vi "DepthProfiling_Proc.vi"(5 "DP_filepath":path=path "", 7 "Params.":variant, 8 "error in (no error)":errorcluster, 9 "Dynamic Params In":refnum<queue>, 10 "Quit_UserEvent":refnum<user-event>, 11 "ControlQueueRef":variant) -> (0 "error out":errorcluster, 2 "Output":variant)   [LabVIEW 2013]
uses:
  Apps_static/ScanParams_SingleLine.ctl
  ProcessMethods/Binning/BinType.ctl
  Files/BinaryHeader.ctl
  ControlDef/QueueRefs.ctl
  ControlDef/LaserCtrl_Method.ctl
  ControlDef/States-AToF.ctl
  <instrlib>/AnalogDiscSDKLv/VIs/DWF_CtrlQueue.ctl
  <instrlib>/AnalogDiscSDKLv/VIs/DWF_State.ctl
  <instrlib>/ESP300/Public/Data/ESP300_State.ctl
  <instrlib>/DG535/Command/DG535_States.ctl
  Hardware/BNC(QuantumComposers)/BNC_States.ctl
  Hardware/FemtoLaser(Legacy)/Laser_Status.ctl
  Hardware/DAQmx(Legacy)/DAQmx_Status.ctl
  ControlDef/Signal.ctl
  ProcessMethods/SignalAverager/ProcessStates.ctl
  Files/WriterState.ctl
  Files/Signal_Segment.ctl
  ControlDef/ProcessingMode.ctl
  Hardware/EPM2000(Legacy)/EPM2K_Status.ctl
  <instrlib>/AnalogDiscSDKLv/VIs/DWF_Signal.ctl
  ControlDef/SampleRateSelector.ctl
  ImagingMS/DirectImaging_State.ctl
  ImagingMS/Imaging_Params.ctl
  ProcessMethods/BioMapConversion/BioMAPWriterCoreParams.ctl
  <vilib>/Utility/error.llb/DialogType.ctl
  <vilib>/Utility/miscctls.llb/LVRowAndColumnTypeDef.ctl
  <vilib>/Analysis/baseanly.llb/Mean (DBL).vi
  UI/Autoscale_Y_Single.vi
  <userlib>/_OpenG.lib/comparison/comparison.llb/I32 Changed__ogtk.vi
  ProcessMethods/Binning/SpectrumBinning.vi
  <instrlib>/ESP300/ESP300.lvlib
  <instrlib>/DG535/SRS_DG535_Lib.lvlib
  <userlib>/Utility/ErrorLog_lib.lvlib
  <vilib>/Analysis/NI_AALBase.lvlib
  <instrlib>/AnalogDiscSDKLv/AnalogDiscSDKLv.lvlib
panel:
  in  "SaveMiddleFile":bool
  out "m/z":dbl=11.0
  out "State":T1(ring)
  in  "Linear/Log":bool
  out "Scan#":i32
  out "PrepScan@Iter 2":i32
  out "PrepScan@Iter":i32
  out "UserEventIter.":i32
  in  "Integration Width (±Da)":dbl=0.5
  in  "m/z (Da)":dbl=11.0
  in  "BinType":T2=enum."ByMass"
  in  "BinWidth":dbl=0.2 min=0.001
  in  "#Layers":i32=1 caption="LayerAverage#" min=1 max=2000 step=1
  in  "Shot#":i32=1 caption="nth of Shot" min=1 max=65535 step=1
  in  "X--":bool
  in  "X++":bool
  in  "Fullscale X":bool
  in  "Fullscale Y":bool
  in  "Y--":bool
  in  "Y++":bool
  out "Depth Profile":dbl[](graph)
  out "Spectra":cluster{"Array":dbl[], dbl[]}(graph)
  in  "Quit":bool
  in  "Cancel":bool
  in  "Peaks of Interest":string[][](table)
  in  "Start":bool
  out "Intensity Graph":dbl[][](graph)
  in  "PeakOI #":i32
  out "MS (Raw)":cluster{"m/z_Array":dbl[], sgl[]}(graph)
  out "Iteration":i32
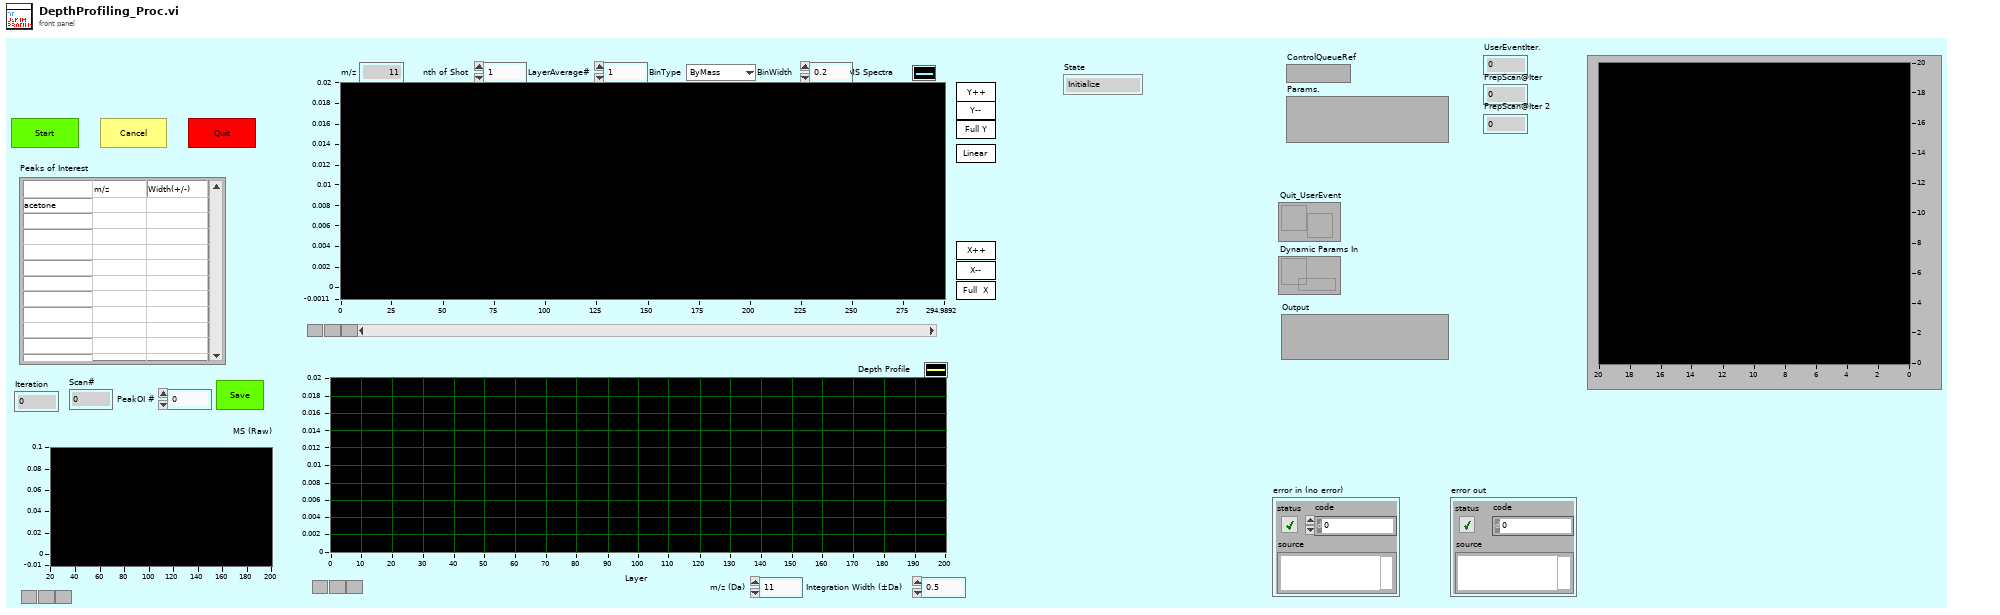
[diagram p1: front panel]
types:
  T1 = enum16{"Initialize", "Open", "PrepScanParams", "WaitData", "Flush", "ScanResult", "CheckEndCondition", "Close", "Quit", "Refresh_Image", "Refresh_Profile", "Refresh_Spectra", "Refresh_RawSpectrum", "SaveMiddleFile", "Save_Image", "SetPeakOI"}
  T2 = typedef "BinType.ctl" = enum16{"ByTime", "ByScreen", "ByMass", "ToUnitMass"}
  T3 = typedef "QueueRefs.ctl" = cluster{"LaserCtrlMethod":T4, "Apps":refnum<queue>, "MainDAQCoreQueue":refnum<queue>, "Micos":refnum<queue>, "ESP300":refnum<queue>, "SMC100":refnum<queue>, "SRS DG535":refnum<queue>, "BNC":refnum<queue>, "SDG_ii":refnum<queue>, "NI-USB_DAQmx":refnum<queue>, "ProcCore_CtrlQueue":refnum<queue>, "WriterCtrl":refnum<queue>, "WriterSIG":refnum<queue>, "Feedback":refnum<queue>, "EPM2000":refnum<queue>, "InfoRef":refnum<vi>, "AppsLock":T5, "ProcCore_SignalQueue":refnum<queue>}
  T4 = typedef "LaserCtrl_Method.ctl" = enum16{"SRS_DG535", "BNC", "SDG_II"}
  T5 = typedef "Semaphore RefNum" = refnum<k1>
  T6 = typedef "ProcessStates.ctl" = enum16{"Initialize", "Normal", "Display", "Write2Buffer", "CalcMzArray", "StartSave", "StopSave", "ConfigChanged", "EndOfLine", "SetFilterParams", "SetGraphsEnable", "SetAcquisitionParams", "ChangeDisplayIncrement", "ChangeRepRate", "SetWriterRef", "Quit", "StartOfLine"}
  T7 = cluster{"Average":i32, "X (Img)":i32, "Y (Img)":i32, "Spectra":sgl[], "Depth":i32, "TickCount":dbl}
  T8 = typedef "BioMAPWriterCoreParams.ctl" = cluster{"File Header":T9, "mzCali.":dbl[], "m/z_Array":dbl[], "SampleRate":T10, "TrigDelay":dbl, "file refnum":refnum<file>, "file path":path, "PeakOI":cluster{"m/z":dbl, "Width(+/-)":dbl}[], "Binning":cluster{"Enable":bool, "BinType":T2, "BinWidth":dbl, "Maximum":dbl, "Minimum":dbl}}
  T9 = typedef "BinaryHeader.ctl" = cluster{"Start Position":dbl[], "StepWidth":dbl[], "Dimension":i32[], "SpecLength":i32}
  T10 = typedef "SampleRateSelector.ctl" = dbl
  T11 = typedef "Imaging_Params.ctl" = cluster{"File Header":T9, "ScanSpeed":dbl, "HighSpeed":dbl, "SampleRate":T10, "Rep.Rate (Hz)":dbl, "TrigDelay":dbl, "mzCali":dbl[], "KeepStill(ms)":u32, "SaveRaw":bool}
  T12 = typedef "DirectImaging_State.ctl" = cluster{"State":enum16{"Initialize", "Open", "PrepScanParams", "WaitData", "Flush", "ScanResult", "CheckEndCondition", "Close", "Quit", "Refresh_Image", "Refresh_Profile", "Refresh_Spectra", "Refresh_RawSpectrum", "SaveMiddleFile", "Save_Image", "SetPeakOI"}, "Para.":variant}
  T13 = cluster{"Save?":bool, "File Header":T9, "Scan#":i32, "ControlRefs":T3, "HighSpeed":dbl, "ScanSpeed":dbl, "SampleRate":T10, "mzCali.":dbl[], "TrigDelay":dbl, "RepRate":dbl, "mzArray":dbl[], "SaveRaw":bool}
  T14 = cluster{"queue out":refnum<queue>, "queue out":refnum<queue>}
  T15 = typedef "Signal.ctl" = cluster{"Command":T6, "Params":variant}
  T16 = typedef "Signal_Segment.ctl" = cluster{"SampleRate":dbl, "TrigDelay":dbl, "SpecLength":dbl, "DAQ_Range":dbl, "Average#":i32, "Position":dbl[], "Spectrum":sgl[], "Calibr.":dbl[], "Pressure":dbl, "Desp_LaserEnergy":dbl, "PI_LaserEnergy":dbl, "Voltages Table":sgl[][], "ProcMode":T17, "Threshold":dbl, "Comment":string, "TickCount":dbl, "Time Stamp":timestamp}
  T17 = typedef "ProcessingMode.ctl" = enum16{"None", "Drop by Threshold", "TDC Simulate", "SetFilter"}
  T18 = typedef "ScanParams_SingleLine.ctl" = cluster{"Line Start":dbl[], "Line End":dbl[], "HighSpeed":dbl, "ScanSpeed":dbl, "KeepStill(ms)":u32, "InstruParams":dbl[]}
  T19 = enum16{"Initialize", "Open", "PrepScanParams", "WaitData", "Flush", "ScanResult", "CheckEndCondition", "Close", "Quit", "Refresh_Image"}
  T20 = cluster{"Average":i32, "X (Img)":i32, "Y (Img)":i32, "Spectra":sgl[], "Depth":i32, "TickCount":dbl}[]
  T21 = typedef "LVRowAndColumnTypeDef.ctl" = cluster{"Row":i32, "Column":i32}
  T22 = typedef "DialogType.ctl" = u16
  T23 = typedef "LVPoint32TypeDef.ctl" = cluster{"Horizontal":i32, "Vertical":i32}
  T24 = typedef "LVRectTypeDef.ctl" = cluster{"Left":i16, "Top":i16, "Right":i16, "Bottom":i16}
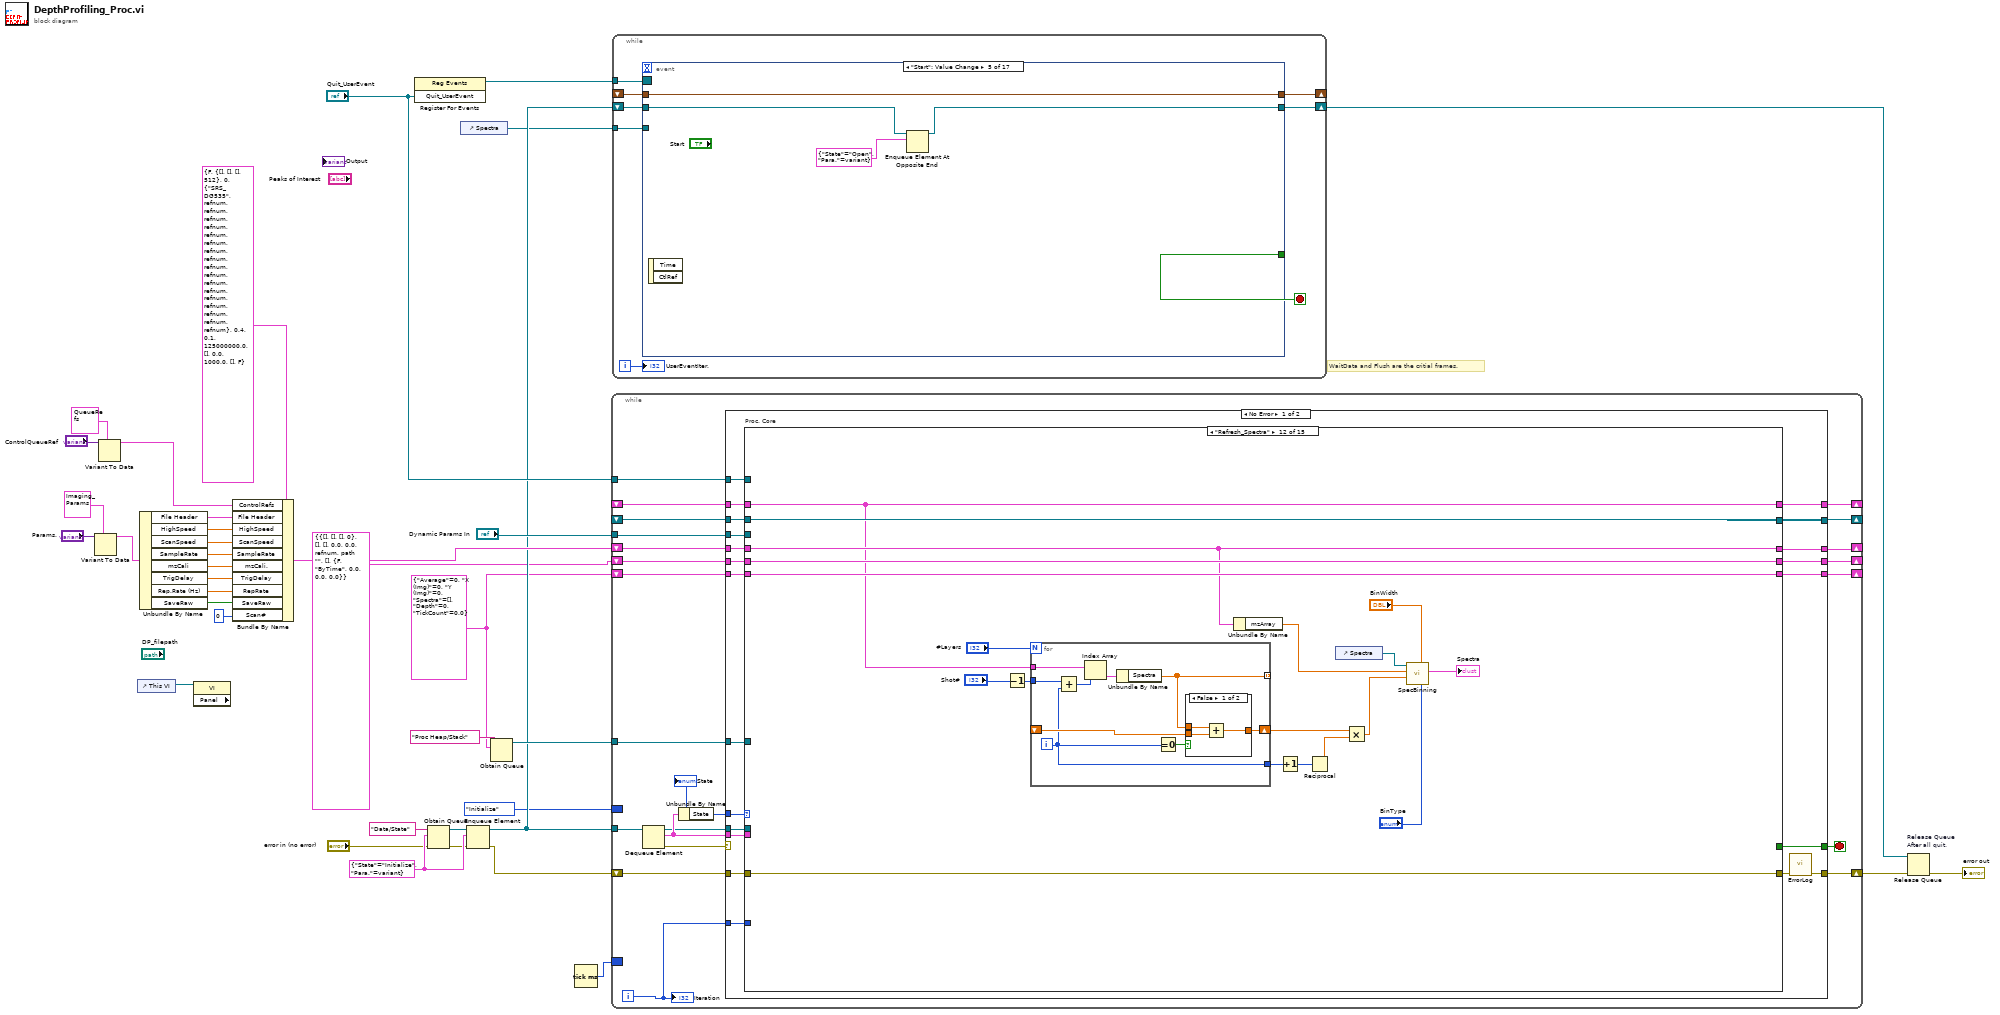
[diagram p0: block diagram]
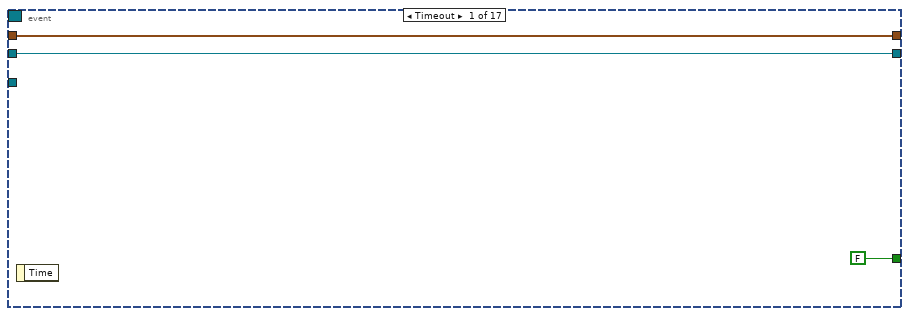
[diagram p2: hidden frame]
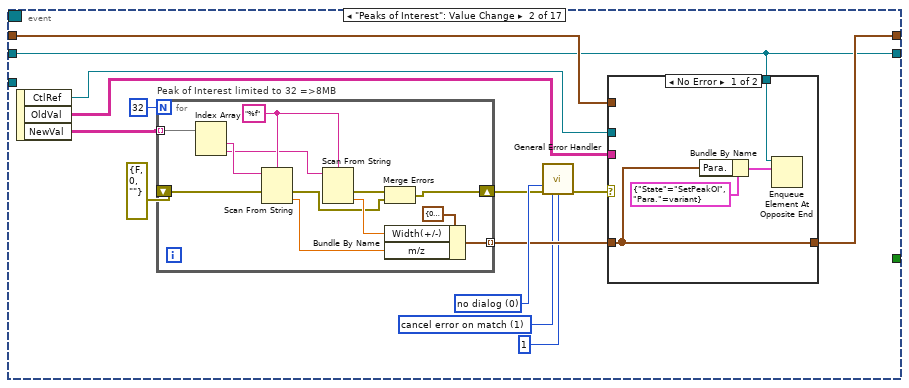
[diagram p3: hidden frame]
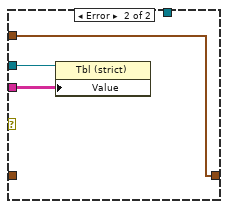
[diagram p4: hidden frame]
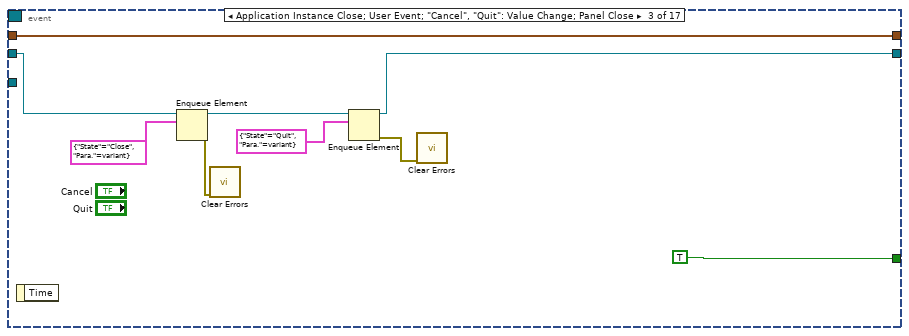
[diagram p5: hidden frame]
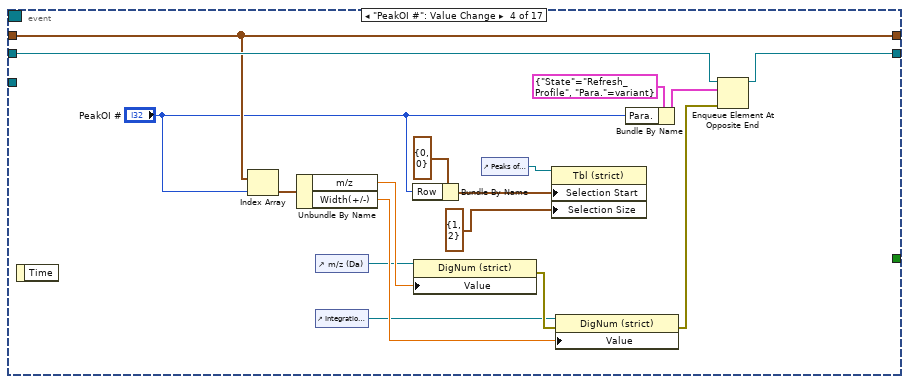
[diagram p6: hidden frame]
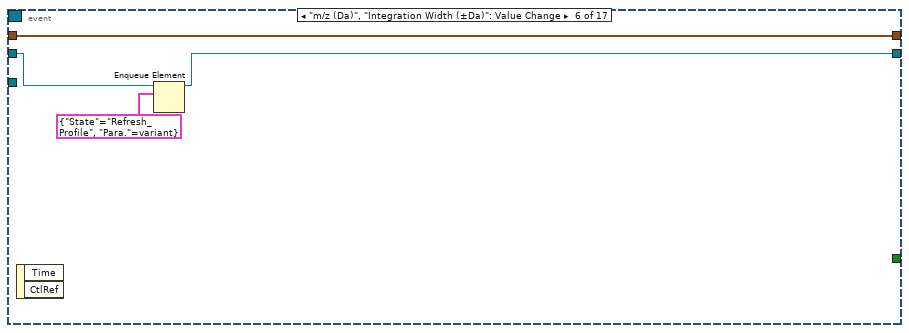
[diagram p7: hidden frame]
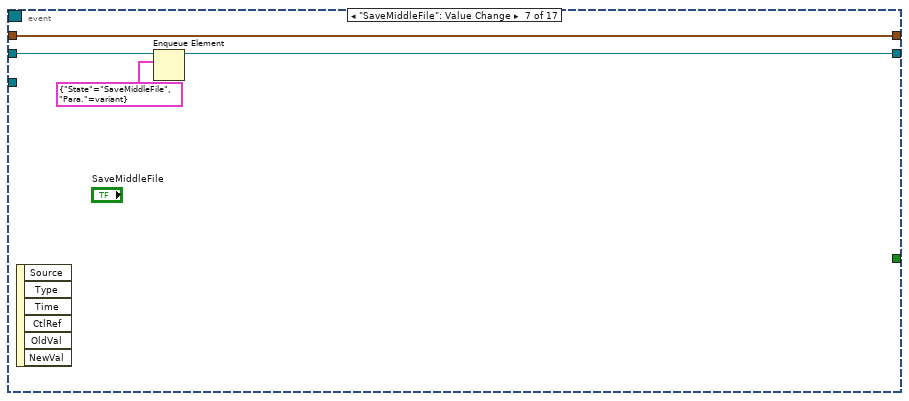
[diagram p8: hidden frame]
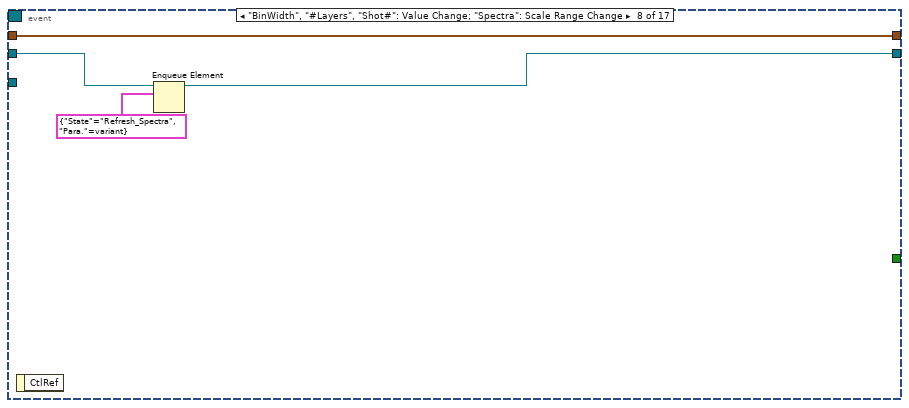
[diagram p9: hidden frame]
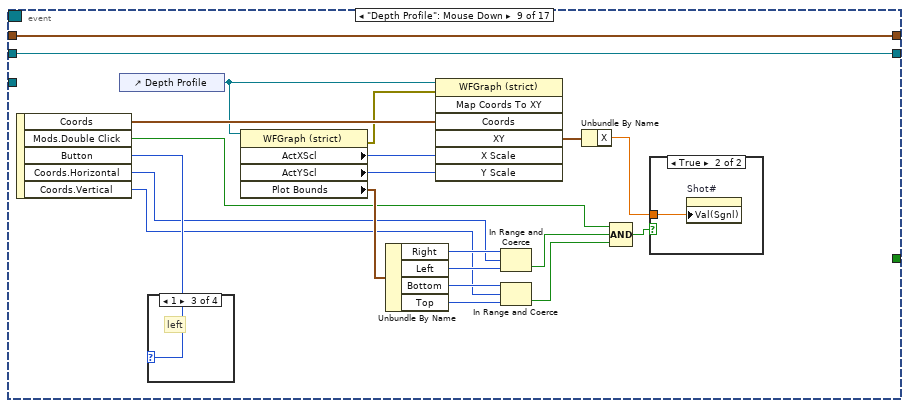
[diagram p10: hidden frame]
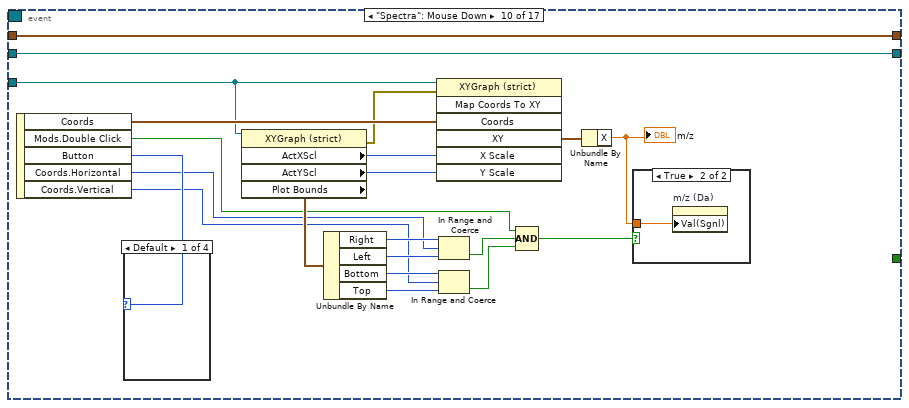
[diagram p15: hidden frame]
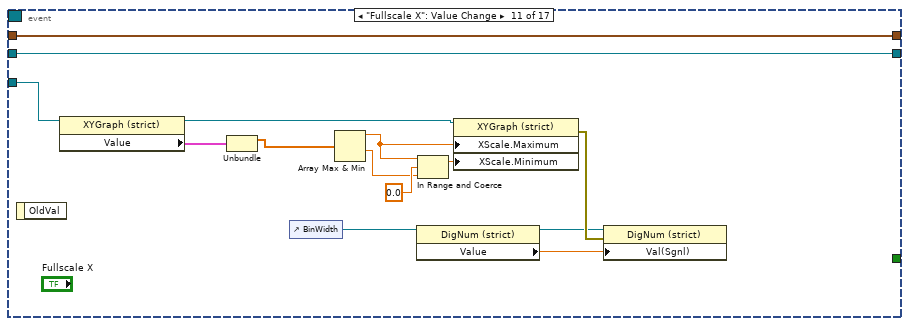
[diagram p20: hidden frame]
diagram:
  w17 = T7 {"Average"=0, "X (Img)"=0, "Y (Img)"=0, "Spectra"=[], "Depth"=0, "TickCount"=0.0} ("output cluster")
  w29 = T12 {"State"=enum."Initialize", "Para."=variant}
  # "WaitData and Flush are the critial frames."
  n1 = Variant To Data(type=T11 {"File Header"={"Start Position"=[], "StepWidth"=[], "Dimension"=[], "SpecLength"=0}, "ScanSpeed"=0.0, "HighSpeed"=0.0, "SampleRate"=0.0, "Rep.Rate (Hz)"=0.0, "TrigDelay"=0.0, "mzCali"=[], "KeepStill(ms)"=0, "SaveRaw"=FALSE} ("BeamProfiling_Params"), Variant="Params.") -> (data=w24:T11)  [unwired: 1 in, 1 out]
  n2 = Variant To Data(type=T3 {"LaserCtrlMethod"=enum."SRS_DG535", "Apps"=refnum, "MainDAQCoreQueue"=refnum, "Micos"=refnum, "ESP300"=refnum, "SMC100"=refnum, "SRS DG535"=refnum, "BNC"=refnum, "SDG_ii"=refnum, "NI-USB_DAQmx"=refnum, "ProcCore_CtrlQueue"=refnum, "WriterCtrl"=refnum, "WriterSIG"=refnum, "Feedback"=refnum, "EPM2000"=refnum, "InfoRef"=refnum, "AppsLock"=refnum, "ProcCore_SignalQueue"=refnum} ("ControlRefs"), Variant="ControlQueueRef") -> (data=w5:T3)  [unwired: 1 in, 1 out]
  n3 = control-ref of="This VI"() -> (w9:refnum<vi>)
  n4 = Unbundle By Name(w24) -> ("File Header"=w23:T9, "HighSpeed"=w22:dbl, "ScanSpeed"=w21:dbl, "SampleRate"=w19:T10, "mzCali"=w11:dbl[], "TrigDelay"=w10:dbl, "Rep.Rate (Hz)"=w2:dbl, "SaveRaw"=w1:bool)
  n5 = property class="VI" props=["Panel"](reference=w9) -> ()  [unwired: 1 in, 3 out]
  n6 = Bundle By Name(cluster=T13 {"Save?"=FALSE, "File Header"={"Start Position"=[], "StepWidth"=[], "Dimension"=[], "SpecLength"=512}, "Scan#"=0, "ControlRefs"={"LaserCtrlMethod"=enum."SRS_DG535", "Apps"=refnum, "MainDAQCoreQueue"=refnum, "Micos"=refnum, "ESP300"=refnum, "SMC100"=refnum, "SRS DG535"=refnum, "BNC"=refnum, "SDG_ii"=refnum, "NI-USB_DAQmx"=refnum, "ProcCore_CtrlQueue"=refnum, "WriterCtrl"=refnum, "WriterSIG"=refnum, "Feedback"=refnum, "EPM2000"=refnum, "InfoRef"=refnum, "AppsLock"=refnum, "ProcCore_SignalQueue"=refnum}, "HighSpeed"=0.4, "ScanSpeed"=0.1, "SampleRate"=125000000.0, "mzCali."=[], "TrigDelay"=0.0, "RepRate"=1000.0, "mzArray"=[], "SaveRaw"=FALSE} ("output cluster"), "ControlRefs"=w5, "File Header"=w23, "HighSpeed"=w22, "ScanSpeed"=w21, "SampleRate"=w19, "mzCali."=w11, "TrigDelay"=w10, "RepRate"=w2, "SaveRaw"=w1, "Scan#"=0) -> (w33:T13)
  n7 = register-events("Quit_UserEvent") -> (reference out=w34:refnum<event-registration>)  [unwired: 2 in, 1 out]
  n8 = Obtain Queue(name (unnamed)="Data/State", element data type=w29, error in (no error)="error in (no error)") -> (queue out=w30:refnum<queue>, error out=w28:errorcluster)  [unwired: 2 in, 1 out]
  n9 = control-ref of="Spectra"() -> (w4:refnum<vi>)
  n10 = Enqueue Element(queue=w30, element=w29, error in (no error)=w28) -> (queue out=w26:refnum<queue>, error out=w18:errorcluster)  [unwired: 1 in, 1 out]
  n11 = Obtain Queue(name (unnamed)="Proc Heap/Stack", element data type=w17) -> (queue out=w38:refnum<queue>)  [unwired: 3 in, 2 out]
  n12 = Tick Count (ms)() -> (millisecond timer value=w16:u32)
  n13 = while {
    shift-right: [w54] -> _
    shift-left: w33 -> [w60]
    tunnel: w26 -> [w59]
    tunnel: w38 -> [w57]
    tunnel: "Dynamic Params In" -> [w51]
    shift-right: [w52] -> _
    shift-left: _ -> [w50]
    shift-right: [w49] -> _
    shift-left: _ -> [w48]
    tunnel: "Quit_UserEvent" -> [w47]
    shift-right: [w45] -> w14
    shift-left: w18 -> [w46]
    shift-right: [w41] -> _
    shift-left: w17 -> [w44]
    shift-right: [w42] -> _
    shift-left: T8 {"File Header"={"Start Position"=[], "StepWidth"=[], "Dimension"=[], "SpecLength"=0}, "mzCali."=[], "m/z_Array"=[], "SampleRate"=0.0, "TrigDelay"=0.0, "file refnum"=refnum, "file path"=path "", "PeakOI"=[], "Binning"={"Enable"=FALSE, "BinType"=enum."ByTime", "BinWidth"=0.0, "Maximum"=0.0, "Minimum"=0.0}} ("output cluster") -> [w43]
    border: w16 -> [_]
    border: ProcessStates."Initialize" -> [_]
    i -> [w39]
    stop <- w53 stop-if-true
    n14 = Dequeue Element(queue=w59) -> (queue out=w55:refnum<queue>, element=w56:T12, error out=w58:errorcluster)  [unwired: 2 in, 1 out]
    n15 = Unbundle By Name(w56) -> ("State"=w40:T1)
    "State" <- w40
    n16 = case shown="No Error" w58 {
      tunnel: w60 -> [w81 w555]
      tunnel: [w80 w555] -> w54
      tunnel: w57 -> [w79 _]
      tunnel: w40 -> [w78 _]
      tunnel: w56 -> [w77 _]
      tunnel: w55 -> [w76 _]
      tunnel: [w75 TRUE] -> w53
      tunnel: [w74 w553] -> w52
      tunnel: w51 -> [w73 _]
      tunnel: w50 -> [w72 w553]
      tunnel: [w71 w552] -> w49
      tunnel: w48 -> [w70 w552]
      tunnel: w47 -> [w69 _]
      tunnel: w46 -> [w68 w551]
      tunnel: [w62 w551] -> w45
      tunnel: w44 -> [w67 w549]
      tunnel: w43 -> [w66 w550]
      tunnel: [w65 w550] -> w42
      tunnel: [w64 w549] -> w41
      tunnel: w39 -> [w61 _]
      frame No Error {
        n17 = case "Proc. Core" shown="\"Refresh_Spectra\"" w78 {
          selector: w78 -> [w85 w157 w194 _ w353 w363 _ _ _ _ _ _ _ _ _]
          tunnel: w81 -> [w95 w132 w200 w220 w328 w368 w385 w404 w410 w441 w459 w481 w523 w542 w548]
          tunnel: [w95 w164 w191 w220 w328 w368 w385 w404 w410 w441 w459 w481 w523 w542 w548] -> w80
          tunnel: w79 -> [_ _ _ w229 w327 _ _ _ w424 _ _ _ _ _ _]
          tunnel: w77 -> [w86 w139 w195 w231 w354 w364 w383 _ _ w435 _ _ _ w530 _]
          tunnel: w76 -> [w87 w158 w185 w232 w355 w365 w384 _ _ w442 _ _ _ _ _]
          tunnel: [_ _ _ _ _ _ _ _ TRUE _ _ _ _ _ _] -> w75
          tunnel: [w103 w133 w192 w230 w336 w362 w382 w402 w423 w436 w454 w479 w511 w541 w547] -> w74
          tunnel: w73 -> [_ _ w197 _ _ _ _ _ w416 _ _ _ _ _ _]
          tunnel: w72 -> [w103 _ w192 w230 w339 w362 w382 w402 w423 w436 w454 w479 w511 w541 w547]
          tunnel: [w102 w153 w190 w224 w352 w361 w381 w394 w422 w440 w455 w493 w522 w540 w546] -> w71
          tunnel: w70 -> [w102 _ w190 w224 w352 w361 w381 w394 w422 w440 w455 w493 w522 w540 w546]
          tunnel: w69 -> [_ _ _ _ _ _ _ _ w421 _ _ _ _ _ _]
          tunnel: w68 -> [w101 w121 w188 w228 _ w360 w379 w393 w412 w439 w467 w492 w509 w539 w545]
          tunnel: [w101 w121 w188 w228 w346 w360 w379 w392 w413 w439 w467 w492 w508 w539 w545] -> w63
          tunnel: w67 -> [w99 w128 w189 w226 w348 w358 w377 _ w415 w437 w465 w490 w521 w538 w543]
          tunnel: w66 -> [w100 w138 w182 w225 w347 w359 w378 w391 w411 w438 w466 w491 w510 w531 w544]
          tunnel: [w97 w145 w182 w225 w347 w359 w378 _ w411 w438 w466 w491 w510 w532 w544] -> w65
          tunnel: [w98 w128 w189 w227 w348 w358 w377 _ w415 w437 w465 w490 w521 w538 w543] -> w64
          tunnel: w61 -> [_ _ w187 _ _ _ _ _ _ _ _ _ _ _ _]
          frame "Initialize" {
            w88 = cluster{"m/z":dbl, "Width(+/-)":dbl}[] [{"m/z"=110.0, "Width(+/-)"=100.0}]  # 10-210 as default range
            w96 = u32[] [0, 0, 12517567, 12320960, 12189888, 12058817, 11927746, 11731139, 11600067, 9175197, 9044125, 11141318, 11010246, 10813639, 10682568, 10551497, 10354890, 10223818, 10092747, 7930019, 7798948, 9633997, 9502926, 9306319, 9175248, 9044176, 8847569, 8716498, 8585427, 6750377, 6619306, 8126677, 7995606, 7798999, 7667927, 7536856, 7340249, 7209178, 7078106, 5505199, 5374128, 6619357, 6488285, 6291678, 6160607, 6029536, 5832929, 5701857, 5570786, 4325557, 4194486, 5112036, 4980965, 4784358, 4653287, 4522215, 4325608, 4194537, 4063466, 3080380, 3014844, 3604716, 3408109, 3277038, 3277038, 3145966, 3014895, 2818288, 2687217, 2556145, 1900738, 1769666, 2097396, 1900789, 1769717, 1638646, 1507575, 1310968, 1179896, 1048825, 721096, 590024, 590075, 393468, 262397, 131326, 255, 1791, 3327, 4863, 5068, 6348, 9471, 11007, 12543, 14079, 15615, 17151, 18687, 20223, 17612, 18636, 25087, 26623, 28159, 29695, 31231, 32767, 34303, 35839, 29900, 31180, 40447, 41983, 43775, 45311, 46847, 48383, 49919, 51455, 42444, 43724, 56063, 57599, 59135, 60671, 62207, 63743, 65535, 65528, 52418, 52413, 65510, 65504, 65498, 65492, 65486, 65480, 65474, 65468, 52369, 52364, 65449, 65443, 65437, 65431, 65425, 65419, 65413, 65407, 52321, 52316, 65389, 65383, 65377, 65371, 65364, 65358, 65352, 65346, 52272, 52267, 65328, 65322, 65316, 65310, 65304, 65298, 65292, 65286, 52224, 314368, 851712, 1244928, 1638144, 2031360, 2424576, 2817792, 3211008, 3604224, 3197952, 3525632, 4783872, 5177088, 5635840, 6029056, 6422272, 6815488, 7208704, 7601920, 6409216, 6736896, 6736896, 8781568, 9174784, 9568000, 9961216, 10354432, 10747648, 11206400, 11599616, 9554944, 9882624, 12779264, 13172480, 13565696, 13958912, 14352128, 14745344, 15138560, 15531776, 12766208, 13093888, 16776960, 16775170, 16773637, 16771847, 16770314, 16768780, 16766991, 16765457, 13411088, 13409810, 16760601, 16758812, 16757278, 16755745, 16753955, 16752422, 16750888, 16749099, 13398052, 13396774, 16744243, 16742704, 16741166, 16739884, 16738345, 16736807, 16735269, 16733730, 13385753, 13384728, 16729371, 16727833, 16726295, 16725012, 16723474, 16721936, 16720397, 16718859, 13373959, 13372677, 16714500, 16712962, 16777215]  # Color table (Rainbow-striped)
            n18 = disable-structure "Wait for user action" shown="Enabled" {
              disable-tunnel: w87 -> [w106 _]
              disable-tunnel: w86 -> [w105 _]
              disable-tunnel: w85 -> [w104 _]
              frame Disabled {
                n19 = Increment(x=w104) -> (x+1=w107:T1)
                n20 = Bundle By Name(cluster=w105, "State"=w107) -> (w108:T12)
                n21 = Enqueue Element(queue=w106, element=w108) -> ()  [unwired: 2 in, 3 out]
              }
              frame Enabled {
              }
            }
            n22 = Unbundle By Name(w95) -> ("File Header.SpecLength"=w90:i32, "File Header"=w84:T9, "mzCali."=w93:dbl[], "SampleRate"=w91:T10, "TrigDelay"=w92:dbl)
            n23 = Subtract(x=w90, y=64) -> (x-y=w82:i32)
            n24 = in-place "Compensate error in float-point number calculation" {
              n25 = in-place-cluster #1(w84) -> ("StepWidth"=w109:dbl[], "Start Position"=w114:dbl[])
              n26 = Index Array(array=w109) -> (element=w113:dbl)  [unwired: 1 in]
              n27 = Multiply(x=w113, y=0.001) -> (x*y=w111:dbl)
              n28 = in-place {
                in-place-border: w111 -> [w116]
                n29 = in-place-array #2(w114, 0) -> (w117:dbl)
                n30 = Subtract(x=w117, y=w116) -> (x-y=w118:dbl)
                n31 = in-place-array #2(w118) -> (w115:dbl[])  [unwired: 1 out]
              }
              n32 = in-place-cluster #1("StepWidth"=w109, "Start Position"=w115) -> (w83:T9)
            }
            n33 = call "CalcMzArray.vi"("TrigDelay"=w92, "Sample Rate"=w91, "Depth"=w82, "mzCali. (a/b/c)"=w93) -> ("mzArray"=w94:dbl[])  [unwired: 7 in]
            n34 = Bundle By Name(cluster=w100, "File Header.SpecLength"=w82, "m/z_Array"=w94, "File Header"=w83, "mzCali."=w93, "SampleRate"=w91, "TrigDelay"=w92, "PeakOI"=w88) -> (w97:T8)
            n35 = Bundle By Name(cluster=w99, "Depth"=w82) -> (w98:T7)
            n36 = property on="Intensity Graph" class="IntGraph (strict)"("Color Table"=w96) -> ()  [unwired: 2 in, 2 out]
          }
          frame "Open" {
            (unwired) T14 {"queue out"=refnum, "queue out"=refnum} ("output cluster")
            w143 = "ActionCallBack" ("name (unnamed)")
            (unwired) 0
            (unwired) cluster{dbl[], dbl[]}[][] []
            # "duplicate??"
            # "8192x32KB*4 = 1GB\n!! attention:\nshould be big"
            n37 = Increment(x=w157) -> (x+1=w159:T1)
            n38 = Bundle By Name(cluster=w139, "State"=w159) -> (w160:T12)
            n39 = Enqueue Element(queue=w158, element=w160) -> ()  [unwired: 2 in, 3 out]
            n40 = Unbundle By Name(w132) -> ("File Header.SpecLength"=w122:i32, "File Header.Dimension"=w131:i32[], "mzCali."=w127:dbl[], "SampleRate"=w126:T10, "TrigDelay"=w125:dbl)
            n41 = call "CalcMzArray.vi"("TrigDelay"=w125, "Sample Rate"=w126, "Depth"=w122, "mzCali. (a/b/c)"=w127) -> ("mzArray"=w123:dbl[])  [unwired: 7 in]
            n42 = Initialize Array(sgl 0.0 ("element"), w122) -> (w135:sgl[])
            n43 = Bundle By Name(cluster=w132, "mzArray"=w123) -> (w124:T13)
            n44 = Bundle By Name(cluster=w128, "Spectra"=w135) -> (w136:T7)
            n45 = Index Array(array=w131, index=2) -> (element=w129:i32)
            n46 = Obtain Queue(max queue size (-1, unlimited)=4192, name (unnamed)="BeamProfiling_Buffer", element data type=T16 {"SampleRate"=0.0, "TrigDelay"=0.0, "SpecLength"=0.0, "DAQ_Range"=0.0, "Average#"=0, "Position"=[], "Spectrum"=[], "Calibr."=[], "Pressure"=0.0, "Desp_LaserEnergy"=0.0, "PI_LaserEnergy"=0.0, "Voltages Table"=[], "ProcMode"=enum."None", "Threshold"=0.0, "Comment"="", "TickCount"=0.0, "Time Stamp"=timestamp(0 s since 1904-01-01)} ("Signal Segment")) -> (queue out=w153:refnum<queue>, error out=w152:errorcluster)  [unwired: 2 in, 1 out]
            n47 = Obtain Queue(name (unnamed)=w143, element data type=w143) -> (queue out=w140:refnum<queue>)  [unwired: 3 in, 2 out]
            n48 = Bundle(cluster=T14 {"queue out"=refnum, "queue out"=refnum}, "queue out"=w153, "queue out"=w140) -> (w144:T14)
            n49 = Initialize Array(w136, w129) -> (w133:T20)
            n50 = Unbundle By Name(w124) -> ("ControlRefs.ProcCore_CtrlQueue"=w154:refnum<queue>)
            n51 = Bundle By Name(cluster=T15 {"Command"=enum."SetWriterRef", "Params"=variant} ("element"), "Command"=ProcessStates."SetWriterRef", "Params"=w144) -> (w162:T15)
            n52 = Enqueue Element "Set Data queue"(queue=w154, element=w162, error in (no error)=w152) -> (queue out=w147:refnum<queue>, error out=w142:errorcluster)  [unwired: 1 in, 1 out]
            n53 = Dequeue Element "Wait DataProc Core Ready"(queue=w140, error in (no error)=w142) -> (error out=w141:errorcluster)  [unwired: 1 in, 3 out]
            n54 = Bundle By Name(cluster=T15 {"Command"=enum."SetWriterRef", "Params"=variant} ("element"), "Command"=ProcessStates."StartSave") -> (w149:T15)
            n55 = Enqueue Element "Start Send Data"(queue=w147, element=w149, error in (no error)=w141) -> (error out=w146:errorcluster)  [unwired: 1 in, 2 out]
            n56 = call <vilib>:"Clear Errors.vi"("error in (no error)"=w146) -> ()  [unwired: 6 in, 1 out]
            n57 = Bundle By Name(cluster=w138, "file path"=path "") -> (w145:T8)
            n58 = Bundle By Name(cluster=w124, "Save?"=FALSE) -> (w164:T13)
          }
          frame "PrepScanParams" {
            # "why timeout ??"
            n59 = Increment(x=w194) -> (x+1=w193:T1)
            n60 = Bundle By Name(cluster=w195, "State"=w193) -> (w184:T12)
            n61 = Unbundle By Name(w200) -> ("Scan#"=w174:i32, "HighSpeed"=w165:dbl, "File Header"=w180:T9, "RepRate"=w177:dbl)  [unwired: 1 out]
            n62 = Increment(x=w174) -> (x+1=w199:i32)
            n63 = Unbundle By Name(w180) -> ("Start Position"=w173:dbl[], "StepWidth"=w169:dbl[], "Dimension"=w179:i32[])
            n64 = Bundle By Name(cluster=w200, "Scan#"=w199) -> (w191:T13)
            n65 = Index Array(array=w179) -> (element #1=w168:i32, element #3=w176:i32)  [unwired: 3 in, 1 out]
            n66 = Quotient & Remainder(x=w174, y=w168) -> (x-y*floor(x/y)=w167:i32, floor(x/y)=w166:i32)
            n67 = Compound Arithmetic op=MULTIPLY(w176, 1000 ("value"), invert w177) -> (w181:dbl)
            n68 = in-place {
              in-place-border: w169 -> [w205]
              in-place-border: w167 -> [w202]
              in-place-border: w166 -> [w201]
              # "Y"
              # "X"
              n69 = in-place-array #3(w173, 0, 1) -> (w210:dbl, w207:dbl)
              n70 = Index Array(array=w205) -> (element #1=w204:dbl, element #2=w203:dbl)  [unwired: 2 in]
              n71 = Multiply(x=w204, y=w202) -> (x*y=w206:dbl)
              n72 = Multiply(x=w203, y=w201) -> (x*y=w209:dbl)
              n73 = Add(x=w210, y=w206) -> (x+y=w211:dbl)
              n74 = Add(x=w207, y=w209) -> (x+y=w208:dbl)
              n75 = in-place-array #3(w211, w208) -> (w172:dbl[])  [unwired: 2 out]
            }
            n76 = Round Toward +Infinity(x=w181) -> (ceil(x): smallest int >= x=w175:dbl)
            n77 = Bundle By Name(cluster=T18 {"Line Start"=[], "Line End"=[], "HighSpeed"=0.0, "ScanSpeed"=0.0, "KeepStill(ms)"=0, "InstruParams"=[]}, "HighSpeed"=w165, "ScanSpeed"=w165, "KeepStill(ms)"=w175, "Line Start"=w172, "Line End"=w172) -> (w196:T18)
            n78 = flat-sequence {
              tunnel: w197 -> [w219]
              tunnel: w196 -> [w218]
              tunnel: w187 -> [w217]
              tunnel: [w217] -> w186
              tunnel: [w214] -> w183
              frame #0 {
                n79 = Enqueue Element "Send scan params"(queue=w219, element=w218, timeout in ms (-1)=1000) -> (timed out?=w214:bool, error out=w215:errorcluster)  [unwired: 1 in, 1 out]
                n80 = call <vilib>:"Clear Errors.vi"("error in (no error)"=w215) -> ()  [unwired: 6 in, 1 out]
              }
            }
            n81 = case shown="False" w183 {
              tunnel: w185 -> [w213 _]
              tunnel: w184 -> [w212 _]
              frame False {
                n82 = Enqueue Element "If not timeout,\ngoto WaitData.\nOtherwise, Idle"(queue=w213, element=w212) -> ()  [unwired: 2 in, 3 out]
              }
              frame True {
              }
            }
            "PrepScan@Iter" <- w187
            "PrepScan@Iter 2" <- w186
          }
          frame "WaitData" {
            # "Data Pre-processor"
            n83 = Dequeue Element "WaitSpectra"(queue=w224, timeout in ms (-1)=1000) -> (element=w223:T16, timed out?=w221:bool)  [unwired: 1 in, 2 out]
            n84 = case shown="False" w221 {
              tunnel: w232 -> [w264 w325]
              tunnel: w231 -> [w263 _]
              tunnel: w229 -> [w262 _]
              tunnel: [w260 w326] -> w227
              tunnel: w226 -> [w259 w326]
              tunnel: w225 -> [w247 _]
              tunnel: w224 -> [w246 _]
              tunnel: w223 -> [w234 _]
              tunnel: w220 -> [w233 _]
              frame False {
                w243 = FALSE  # True for missing EOL (Legacy)
                # "TODO:  Remove average forcing 1 to sum true average#!!"
                n85 = Unbundle By Name(w233) -> ("ControlRefs.WriterSIG"=w235:refnum<queue>)  [unwired: 1 out]
                n86 = Unbundle By Name(w247) -> ("File Header.Start Position"=w250:dbl[], "File Header.StepWidth"=w251:dbl[])
                n87 = Unbundle By Name(w234) -> ("TickCount"=w237:dbl, "Position"=w252:dbl[], "Spectrum"=w241:sgl[], "Average#"=w239:i32, "Comment"=w238:string)
                n88 = String Subset(string=w238, length (rest)=2 ("length (rest)")) -> ()  [unwired: 1 in, 1 out]
                n89 = Type Cast(type=ProcessStates."StartOfLine", x=w238) -> (*(type *) &x=w249:T6)
                n90 = feedback #4() -> (w248:T6)
                n91 = feedback-in #4(w249) -> ()
                n92 = case shown="True" FALSE {
                  tunnel: w234 -> [_ w266]
                  tunnel: w235 -> [_ w265]
                  frame False {
                  }
                  frame True {
                    n93 = Enqueue Element(queue=w265, element=w266) -> ()  [unwired: 2 in, 3 out]
                  }
                }
                n94 = Multiply(x=w241, y=w239) -> (x*y=w240:sgl[])
                n95 = case "Average Spectra in a single pixel" shown="Default" w249 {
                  tunnel: w264 -> [w285 w291 w321]
                  tunnel: w262 -> [w284 w289 w319]
                  tunnel: w263 -> [_ w290 w320]
                  tunnel: w259 -> [_ _ w296]
                  tunnel: [_ _ w307] -> w260
                  tunnel: [_ _ w292] -> w253
                  tunnel: w240 -> [_ _ w292]
                  tunnel: w252 -> [_ _ w306]
                  tunnel: w251 -> [_ _ w305]
                  tunnel: w250 -> [_ _ w304]
                  tunnel: w248 -> [_ _ w302]
                  tunnel: [_ _ w297] -> w245
                  tunnel: w239 -> [_ _ w298]
                  tunnel: w237 -> [_ _ w295]
                  frame "EndOfLine" {
                    # "Not idea solution,\nWhy this? Did not I handled this in flush??"
                    # "End of Line"
                    n96 = Get Queue Status(queue=w284) -> (queue out=w283:refnum<queue>, # elements in queue=w282:i32)  [unwired: 2 in, 6 out]
                    n97 = Less?(x=w282, y=5) -> ()  [unwired: 1 out]
                    n98 = case shown="False" FALSE {
                      tunnel: w283 -> [_ w288]
                      tunnel: [T12 {"State"=enum."Flush", "Para."=variant} ("element") T12 {"State"=enum."WaitData", "Para."=variant} ("element")] -> w280
                      frame False {
                      }
                      frame True {
                        n99 = Flush Queue(queue=w288) -> ()  [unwired: 1 in, 3 out]
                      }
                    }
                    n100 = Enqueue Element At Opposite End(queue=w285, element=w280) -> ()  [unwired: 2 in, 3 out]
                  }
                  frame "StartOfLine" {
                    # "New Line"
                    n101 = Enqueue Element "Implied \"WaitData\""(queue=w291, element=w290) -> ()  [unwired: 2 in, 3 out]
                    n102 = Flush Queue(queue=w289) -> ()  [unwired: 1 in, 3 out]
                  }
                  frame Default {
                    # "Normal Spectra"
                    n103 = Index Array(array=w304) -> (element #1=w314:dbl, element #2=w315:dbl)  [unwired: 2 in]
                    n104 = Index Array(array=w305) -> (element #1=w316:dbl, element #2=w317:dbl)  [unwired: 2 in]
                    n105 = Index Array(array=w306) -> (element #1=w301:dbl, element #2=w318:dbl)  [unwired: 2 in]
                    n106 = Enqueue Element "Implied \"WaitData\""(queue=w321, element=w320) -> ()  [unwired: 2 in, 3 out]
                    n107 = Subtract "Y"(x=w318, y=w315) -> (x-y=w311:dbl)
                    n108 = Subtract "X"(x=w301, y=w314) -> (x-y=w312:dbl)
                    n109 = Divide(x=w311, y=w317) -> (x/y=w310:dbl)
                    n110 = Divide(x=w312, y=w316) -> (x/y=w313:dbl)
                    n111 = Round Toward -Infinity(1:w313) -> (0:w308:dbl)
                    n112 = Round Toward -Infinity(1:w310) -> (0:w309:dbl)
                    n113 = To Long Integer(number=w308) -> (32bit integer=w299:i32)
                    n114 = To Long Integer(number=w309) -> (32bit integer=w300:i32)
                    n115 = call-poly <userlib>:"Data Changed__ogtk.vi"("I32"=w300) -> ("Changed"=w297:bool)
                    n116 = call-poly <userlib>:"Data Changed__ogtk.vi"("I32"=w299) -> ("Changed"=w303:bool)
                    n117 = Bundle By Name(cluster=w296, "TickCount"=w295, "X (Img)"=w299, "Y (Img)"=w300, "Spectra"=w292, "Average"=w298) -> (w307:T7)
                    n118 = Or(x=w297, y=w303) -> ()  [unwired: 1 out]
                    n119 = Not Equal?(x=ProcessStates."StartOfLine", y=w302) -> (x != y?=w293:bool)
                    n120 = case shown="True" w293 {
                      tunnel: w319 -> [_ w323]
                      tunnel: w307 -> [_ w322]
                      frame False {
                      }
                      frame True {
                        n121 = Enqueue Element ("Push previous to stack")(queue=w323, element=w322) -> ()  [unwired: 2 in, 3 out]
                      }
                    }
                  }
                }
                n122 = Tick Count (ms)() -> (millisecond timer value=w255:u32)
                n123 = Less?(x=u32 50, y=w255) -> (x < y?=w256:bool)
                n124 = feedback #5() -> (w257:u32)
                n125 = case "raw MS refresh" shown="True" w256 {
                  tunnel: w253 -> [_ w277]
                  tunnel: w255 -> [_ w278]
                  tunnel: [w273 w278] -> w258
                  tunnel: w257 -> [w273 _]
                  tunnel: w247 -> [_ w275]
                  frame False {
                  }
                  frame True {
                    n126 = Unbundle By Name(w275) -> ("m/z_Array"=w276:dbl[])
                    n127 = Bundle("m/z_Array"=w276, w277) -> (→"MS (Raw)":cluster{"m/z_Array":dbl[], sgl[]})  [unwired: 1 in]
                  }
                }
                n128 = feedback-in #5(w258) -> ()
                n129 = And(x=w245, y=w243) -> (x .and. y?=w244:bool)
                n130 = case "For Legacy Format" shown="True" w244 {
                  tunnel: w246 -> [_ w272]
                  frame False {
                  }
                  frame True {
                    n131 = Type Cast(type="", x=ProcessStates."EndOfLine") -> (*(type *) &x=w271:string)
                    n132 = Bundle By Name(cluster=T16 {"SampleRate"=-1.0, "TrigDelay"=0.0, "SpecLength"=0.0, "DAQ_Range"=0.0, "Average#"=0, "Position"=[], "Spectrum"=[], "Calibr."=[], "Pressure"=-1.0, "Desp_LaserEnergy"=-1.0, "PI_LaserEnergy"=-1.0, "Voltages Table"=[], "ProcMode"=enum."None", "Threshold"=-1.0, "Comment"="", "TickCount"=0.0, "Time Stamp"=timestamp(0 s since 1904-01-01)} ("Value"), "Comment"=w271) -> (w267:T16)
                    n133 = Enqueue Element At Opposite End(queue=w272, element=w267) -> ()  [unwired: 2 in, 3 out]
                  }
                }
              }
              frame True {
                # "this frame can be optimized, to minimize unnecessary flushing"
                n134 = Enqueue Element(queue=w325, element=T12 {"State"=enum."Flush", "Para."=variant}) -> ()  [unwired: 2 in, 3 out]
              }
            }
          }
          frame "Flush" {
            # "Data formater/organizer"
            n135 = Increment(x=w353) -> (x+1=w356:T1)
            n136 = Bundle By Name(cluster=w354, "State"=w356) -> (w357:T12)
            n137 = Enqueue Element(queue=w355, element=w357) -> (queue out=w345:refnum<queue>, error out=w343:errorcluster)  [unwired: 2 in, 1 out]
            n138 = property on="PeakOI #" class="DigNum (strict)"() -> ("Value"=w340:i32)  [unwired: 2 in, 2 out]
            n139 = Bundle By Name(cluster=T12 {"State"=enum."Refresh_Image", "Para."=variant} ("element"), "Para."=w340) -> (w341:T12)
            n140 = Enqueue Element(queue=w345, element=w341, error in (no error)=w343) -> (error out=w344:errorcluster)  [unwired: 1 in, 2 out]
            n141 = control-ref of="This VI"() -> (w351:refnum<vi>)
            n142 = property class="VI"(reference=w351, error in=w344, "FP:RunTransparently"=FALSE ("Front Panel Window:Run VI Transparently"), "FP:Transparency"=u8 0 ("Front Panel Window:Transparency")) -> (error out=w338:errorcluster)  [unwired: 1 out]
            n143 = Unbundle By Name(w328) -> ("File Header.Dimension"=w335:i32[], "RepRate"=w333:dbl)
            n144 = Index Array(array=w335, index=2) -> (element=w330:i32)
            n145 = Select(t=500, s=FALSE, f=w330) -> (s? t:f=w329:i32)
            n146 = call "DepthProfileWriteCore.vi"("Buffer In"=w339, "error in"=w338, "RepRate (Hz)"=w333, "Total_Depth (shots)"=w329, "pre-Processed_Buffer"=w327) -> ("error out"=w337:errorcluster, "Buffer Out"=w336:T20)  [unwired: 5 in]
            n147 = call <vilib>:"General Error Handler.vi"("error in (no error)"=w337) -> ("error out"=w346:errorcluster)  [unwired: 10 in, 4 out]
          }
          frame "ScanResult" {
            n148 = Increment(x=w363) -> (x+1=w366:T1)
            n149 = Bundle By Name(cluster=w364, "State"=w366) -> (w367:T12)
            n150 = Enqueue Element(queue=w365, element=w367) -> ()  [unwired: 2 in, 3 out]
          }
          frame "CheckEndCondition" {
            n151 = Unbundle By Name(w385) -> ("Scan#"=w386:i32, "File Header.Dimension"=w387:i32[])
            "Scan#" <- w386
            n152 = Index Array(array=w387) -> (element #1=w372:i32, element #2=w371:i32)  [unwired: 2 in]
            n153 = Increment(x=w386) -> (x+1=w369:i32)
            n154 = Multiply(x=w372, y=w371) -> (x*y=w370:i32)
            n155 = Greater Or Equal? "Determine end condition"(x=w369, y=w370) -> (x >= y?=w373:bool)
            n156 = Select(t=T19."Close" ("State"), s=w373, f=T19."PrepScanParams" ("State")) -> (s? t:f=w374:T19)
            n157 = Bundle By Name(cluster=w383, "State"=w374) -> (w380:T12)
            n158 = Enqueue Element(queue=w384, element=w380) -> ()  [unwired: 2 in, 3 out]
          }
          frame "Close" {
            n159 = Unbundle By Name(w391) -> ("file path"=w388:path)
            n160 = Not Equal?(x=w388, y=path "" ("file path")) -> (x != y?=w390:bool)
            n161 = case shown="True" w390 {
              tunnel: w393 -> [w408 w409]
              tunnel: w391 -> [_ _]
              tunnel: [w408 w409] -> w392
              frame False {
              }
              frame True {
                # "Add write files VIs here"
              }
            }
            n162 = Unbundle By Name(w404) -> ("ControlRefs.ProcCore_CtrlQueue"=w399:refnum<queue>, "ControlRefs.WriterSIG"=w403:refnum<queue>)
            n163 = Bundle By Name(cluster=T15 {"Command"=enum."SetWriterRef", "Params"=variant} ("element"), "Command"=ProcessStates."StopSave") -> (w398:T15)
            n164 = Bundle By Name(cluster=T15 {"Command"=enum."SetWriterRef", "Params"=variant} ("element"), "Command"=ProcessStates."SetWriterRef", "Params"=w403) -> (w406:T15)
            n165 = Enqueue Element(queue=w399, element=w398) -> (queue out=w397:refnum<queue>, error out=w396:errorcluster)  [unwired: 2 in, 1 out]
            n166 = Enqueue Element(queue=w397, element=w406, error in (no error)=w396) -> (error out=w395:errorcluster)  [unwired: 1 in, 2 out]
            n167 = call <vilib>:"Clear Errors.vi"("error in (no error)"=w395) -> ()  [unwired: 6 in, 1 out]
          }
          frame "Quit" {
            n168 = disable-structure shown="Enabled" {
              disable-tunnel: w416 -> [w431 _]
              disable-tunnel: w410 -> [w427 _]
              frame Enabled {
                # "Bad solution: have upper level jump out wait queue"
                n169 = Unbundle By Name(w427) -> ("HighSpeed"=w426:dbl)
                n170 = Bundle By Name(cluster=T18 {"Line Start"=[], "Line End"=[], "HighSpeed"=0.0, "ScanSpeed"=0.0, "KeepStill(ms)"=0, "InstruParams"=[]} ("element"), "HighSpeed"=w426, "ScanSpeed"=w426) -> (w428:T18)
                n171 = Enqueue Element(queue=w431, element=w428) -> (error out=w429:errorcluster)  [unwired: 2 in, 2 out]
                n172 = call <vilib>:"Clear Errors.vi"("error in (no error)"=w429) -> ()  [unwired: 6 in, 1 out]
              }
              frame Disabled {
              }
            }
            n173 = Release Queue(queue=w424, error in (no error)=w412) -> (error out=w414:errorcluster)  [unwired: 1 in, 2 out]
            n174 = Generate User Event(user event=w421, event data cluster=cluster{bool} {TRUE} ("event data")) -> (user event out=w419:refnum<user-event>, error out=w418:errorcluster)  [unwired: 2 in]
            n175 = Destroy User Event(user event=w419, error in=w418) -> (error out=w417:errorcluster)
            n176 = Merge Errors(w417, w414) -> (w413:errorcluster)
          }
          frame "Refresh_Image" {
            # "Call command has to be push to the end not start of the queue."
            n177 = Unbundle By Name(w435) -> ("Para."=w434:variant)
            n178 = Variant To Data(type=1 ("PeakOI #"), Variant=w434) -> (data=w432:i32)  [unwired: 1 in, 1 out]
            n179 = disable-structure shown="Disabled" {
              disable-tunnel: w442 -> [w451 _]
              frame Disabled {
                n180 = Get Queue Status(queue=w451) -> (# pending remove=w450:i32)  [unwired: 2 in, 7 out]
                n181 = Equal To 0?(x=w450) -> (x = 0?=w449:bool)
                n182 = case shown="True" w449 {
                  frame False {
                  }
                  frame True {
                    n183 = One Button Dialog(message="Internal error:\nNothing in queue while refresh curves.") -> ()  [unwired: 1 in, 1 out]
                  }
                }
              }
              frame Enabled {
              }
            }
            n184 = disable-structure shown="Disabled" {
              disable-tunnel: w436 -> [w448 _]
              disable-tunnel: w432 -> [w445 _]
              frame Disabled {
                n185 = Array Subset(array=w448, index (dim 2)=w445, length (dim 2)=1 ("length")) -> (w447:T20)  [unwired: 4 in]
                n186 = Array Size(array=w447) -> ()  [unwired: 1 out]
                n187 = control-ref of="Intensity Graph"() -> (w444:refnum<vi>)
                n188 = property class="IntGraph (strict)" props=["ZScale", "Maximum", "ZScale", "Minimum"](reference=w444, "ZScale.Minimum"=0.0 ("Z Scale.Range:Minimum")) -> ()  [unwired: 2 in, 2 out]
              }
              frame Enabled {
              }
            }
          }
          frame "Refresh_Profile" {
            n189 = Unbundle By Name(w459) -> ("mzArray"=w458:dbl[])
            n190 = Subtract(x="m/z (Da)", y="Integration Width (±Da)") -> (x-y=w463:dbl)
            n191 = Add(x="m/z (Da)", y="Integration Width (±Da)") -> (x+y=w464:dbl)
            n192 = Threshold 1D Array(2:w463, 3:w458) -> (0:w460:dbl)  [unwired: 1 in]
            n193 = Round Toward -Infinity(1:w460) -> (0:w462:dbl)
            n194 = Threshold 1D Array(1:w462, 2:w464, 3:w458) -> (0:w461:dbl)
            n195 = for {
              tunnel: w454 -> [w474] mode=indexing
              tunnel: [w470] -> w453 mode=indexing
              tunnel: w461 -> [w469]
              tunnel: w462 -> [w468]
              n196 = Unbundle By Name(w474) -> ("Spectra"=w473:sgl[])
              n197 = Subtract(x=w469, y=w468) -> (x-y=w472:dbl)
              n198 = Array Subset(array=w473, index=w468, length=w472) -> (w471:sgl[])
              n199 = call-poly <vilib>:"Mean.vi"("X"=w471) -> ("mean"=w470:dbl)  [unwired: 1 out]
            }
            "Depth Profile" <- w453
          }
          frame "Refresh_Spectra" {
            n200 = Decrement(x="Shot#") -> (x-1=w488:i32)
            n201 = for {
              N: "#Layers" -> [_]
              tunnel: w479 -> [w502]
              tunnel: w488 -> [w500]
              shift-right: [w498] -> w484
              shift-left: _ -> [w497]
              tunnel: [w495] -> w486
              tunnel: [w494] -> _ mode=indexing
              i -> [w495]
              n202 = Add(x=w500, y=w495) -> (x+y=w499:i32)
              n203 = Index Array(array=w502, index=w499) -> (element=w501:T7)
              n204 = Unbundle By Name(w501) -> ("Spectra"=w494:sgl[])
              n205 = Equal To 0?(x=w495) -> (x = 0?=w496:bool)
              n206 = case shown="False" w496 {
                tunnel: [w505 w506] -> w498
                tunnel: w497 -> [w504 _]
                tunnel: w494 -> [w503 w506]
                frame False {
                  n207 = Add(x=w503, y=w504) -> (x+y=w505:sgl[])
                }
                frame True {
                }
              }
            }
            n208 = Unbundle By Name(w481) -> ("mzArray"=w480:dbl[])
            n209 = Increment(x=w486) -> (x+1=w487:i32)
            n210 = Reciprocal(x=w487) -> (1/x=w485:dbl)
            n211 = control-ref of="Spectra"() -> (w475:refnum<vi>)
            n212 = Multiply(x=w484, y=w485) -> (x*y=w489:dbl[])
            n213 = call-poly "SpecBinning.vi"("BinType"="BinType", "BinWidth"="BinWidth", "Signal"=w489, "m/z Array"=w480, "GraphRef."=w475) -> ("BinnedSpectrum"=→"Spectra":cluster{"m/z Array":dbl[], "Signal":dbl[]})  [unwired: 5 in, 1 out]
          }
          frame "SaveMiddleFile" {
            n214 = call <vilib>:"Dflt Data Dir.vi"() -> ("App:Default Data Directory"=w507:path)
            n215 = feedback #6(w507) -> (w513:path)
            n216 = Strip Path(path=w513) -> (stripped path=w517:path, name=w516:string)
            n217 = call "File Dialog"("start path"=w517, "default name"=w516, "error in"=w509, "pattern (all files)"="*.dp.bin", "pattern label"="Depth Profile File") -> ("selected path"=w515:path, "cancelled"=w520:bool, "error out"=w512:errorcluster)  [unwired: 7 in, 1 out]
            n218 = case shown="False" w520 {
              tunnel: w515 -> [w527 _]
              tunnel: [w527 w529] -> w514
              tunnel: w513 -> [_ w529]
              tunnel: w512 -> [w526 _]
              tunnel: w511 -> [w528 _]
              tunnel: [w525 _] -> w508
              tunnel: w510 -> [w524 _]
              frame False {
                n219 = call "DepthProfileFormat_Writer.vi"("error in"=w526, "DepthProfilingArray"=w528, "AcquisitionParams."=w524, "depth profile file path"=w527) -> ("error out"=w525:errorcluster)  [unwired: 7 in]
              }
              frame True {
              }
            }
            n220 = feedback-in #6(w514) -> ()
          }
          frame "SetPeakOI" {
            n221 = Unbundle By Name(w531) -> ("PeakOI"=w537:cluster{"m/z":dbl, "Width(+/-)":dbl}[])
            n222 = Unbundle By Name(w530) -> ("Para."=w533:variant)
            n223 = Variant To Data(type=w537, Variant=w533) -> (data=w535:cluster{"m/z":dbl, "Width(+/-)":dbl}[], error out=w534:errorcluster)  [unwired: 1 in]
            n224 = Select(t=w537, s=w534, f=w535) -> (s? t:f=w536:cluster{"m/z":dbl, "Width(+/-)":dbl}[])
            n225 = Bundle By Name(cluster=w531, "PeakOI"=w536) -> (w532:T8)
          }
          frame Default {
            # "Doing nothing, if frame not supported by this processing vi"
          }
        }
        n226 = call <userlib>:"ErrorLog.vi"("error in (no error)"=w63) -> ("error out"=w62:errorcluster)  [unwired: 10 in]
      }
      frame Error {
      }
    }
    "Iteration" <- w39
  }
  n227 = while {
    tunnel: w34 -> [w561]
    shift-right: [w560] -> w12
    shift-left: w26 -> [w563]
    shift-right: [w559] -> _
    shift-left: _ -> [w558]
    tunnel: w4 -> [w557]
    i -> [w556]
    stop <- w562 stop-if-true
    n228 = event shown="[4] \"Start\": Value Change" {
      selector: w561 -> [_ _ _ _ _ _ _ _ _ _ _ _ _ _ _ _ _]
      dyn-events: _ -> [_ _ _ _ _ _ _ _ _ _ _ _ _ _ _ _ _]
      timeout: _ -> [_ _ _ _ _ _ _ _ _ _ _ _ _ _ _ _ _]
      tunnel: w563 -> [w565 w568 w605 w622 w629 w631 w635 w640 w659 w681 w685 w699 w706 w708 w726 w744 w773]
      tunnel: [FALSE _ TRUE _ _ _ _ _ _ _ _ _ _ _ _ _ _] -> w562
      tunnel: [w565 w568 w601 w623 w628 w630 w634 w640 w659 w681 w685 w699 w706 w708 w726 w744 w773] -> w560
      tunnel: [w564 w569 w600 w617 w627 w633 w637 w639 w661 w683 w698 w701 w707 w725 w743 w765 w794] -> w559
      tunnel: w558 -> [w564 w570 w600 w617 w627 w633 w637 w639 w661 w683 w698 w701 w707 w725 w743 w765 w794]
      tunnel: w557 -> [_ _ _ _ _ _ _ _ _ w675 w687 w700 _ w710 w728 w745 w774]
      event Timeout {
        n229 = event-data() -> ()  [unwired: 1 in, 1 out]
      }
      event "Peaks of Interest": Value Change {
        w580 = T22 0 items=["no dialog", "OK message", "continue or stop message", "OK message + warnings", "continue/stop + warnings"] ("type of dialog (OK msg:1)")
        w577 = 1 items=["no exception", "cancel error on match", "set error on match"] ("[exception action] (none:0)")
        n230 = event-data() -> ("CtlRef"=w567:refnum<vi>, "OldVal"=w571:string[][], "NewVal"=w572:string[][])  [unwired: 1 in]
        n231 = for "Peak of Interest limited to 32 =>8MB" {
          N: 32 -> [_]
          tunnel: w572 -> [w592] mode=indexing
          shift-right: [w584] -> w576
          shift-left: errorcluster {"status"=FALSE, "code"=0, "source"=""} ("error IO") -> [w586]
          tunnel: [w585] -> w578 mode=indexing
          w591 = "%f" ("format string")
          n232 = Index Array(array=w592) -> (element #1=w582:string, element #2=w581:string)  [unwired: 2 in]
          n233 = Scan From String(format string=w591, input string=w582, error in=w586) -> (error out=w583:errorcluster, output 1=w588:dbl)  [unwired: 2 in, 2 out]
          n234 = Scan From String(format string=w591, input string=w581) -> (error out=w587:errorcluster, output 1=w589:dbl)  [unwired: 3 in, 2 out]
          n235 = Merge Errors(w587, w583) -> (w584:errorcluster)
          n236 = Bundle By Name(cluster=cluster{"m/z":dbl, "Width(+/-)":dbl} {"m/z"=0.0, "Width(+/-)"=0.0} ("Peak-Of-Interest"), "Width(+/-)"=w589, "m/z"=w588) -> (w585:cluster{"m/z":dbl, "Width(+/-)":dbl})
        }
        n237 = call <vilib>:"General Error Handler.vi"("type of dialog (OK msg:1)"=w580, "error in (no error)"=w576, "[exception action] (none:0)"=w577, "[exception code]"=1) -> ("error out"=w575:errorcluster)  [unwired: 7 in, 4 out]
        n238 = case shown="No Error" w575 {
          tunnel: w571 -> [_ w599]
          tunnel: [w594 w598] -> w569
          tunnel: w578 -> [w594 _]
          tunnel: w570 -> [_ w598]
          tunnel: w568 -> [w593 _]
          tunnel: w567 -> [_ w597]
          frame No Error {
            n239 = Bundle By Name(cluster=T12 {"State"=enum."SetPeakOI", "Para."=variant} ("element"), "Para."=w594) -> (w595:T12)
            n240 = Enqueue Element At Opposite End(queue=w593, element=w595) -> ()  [unwired: 2 in, 3 out]
          }
          frame Error {
            n241 = property on="Property Node" class="Tbl (strict)"(reference=w597, "Value"=w599) -> ()  [unwired: 1 in, 2 out]
          }
        }
      }
      event Application Instance Close; User Event; "Cancel", "Quit": Value Change; Panel Close {
        n242 = event-data() -> ()  [unwired: 1 in, 1 out]
        n243 = Enqueue Element(queue=w605, element=T12 {"State"=enum."Close", "Para."=variant}) -> (queue out=w606:refnum<queue>, error out=w604:errorcluster)  [unwired: 2 in, 1 out]
        n244 = call <vilib>:"Clear Errors.vi"("error in (no error)"=w604) -> ()  [unwired: 6 in, 1 out]
        n245 = Enqueue Element(queue=w606, element=T12 {"State"=enum."Quit", "Para."=variant}) -> (queue out=w601:refnum<queue>, error out=w607:errorcluster)  [unwired: 2 in, 1 out]
        n246 = call <vilib>:"Clear Errors.vi"("error in (no error)"=w607) -> ()  [unwired: 6 in, 1 out]
      }
      event "PeakOI #": Value Change {
        n247 = event-data() -> ()  [unwired: 1 in, 1 out]
        n248 = Index Array(array=w617, index="PeakOI #") -> (element=w615:cluster{"m/z":dbl, "Width(+/-)":dbl})
        n249 = Unbundle By Name(w615) -> ("m/z"=w614:dbl, "Width(+/-)"=w613:dbl)
        n250 = control-ref of="m/z (Da)"() -> (w610:refnum<vi>)
        n251 = control-ref of="Integration Width (±Da)"() -> (w609:refnum<vi>)
        n252 = Bundle By Name(cluster=T21 {"Row"=0, "Column"=0} ("Selection Start"), "Row"="PeakOI #") -> (w620:T21)
        n253 = property class="DigNum (strict)"(reference=w610, "Value"=w614) -> (error out=w612:errorcluster)  [unwired: 1 in, 1 out]
        n254 = control-ref of="Peaks of Interest"() -> (w618:refnum<vi>)
        n255 = property on="Property Node" class="Tbl (strict)"(reference=w618, "Selection Start"=w620, "Selection Size"=T21 {"Row"=1, "Column"=2}) -> ()  [unwired: 1 in, 2 out]
        n256 = property class="DigNum (strict)"(reference=w609, error in=w612, "Value"=w613) -> (error out=w611:errorcluster)  [unwired: 1 out]
        n257 = Bundle By Name(cluster=T12 {"State"=enum."Refresh_Profile", "Para."=variant} ("element"), "Para."="PeakOI #") -> (w624:T12)
        n258 = Enqueue Element At Opposite End(queue=w622, element=w624, error in (no error)=w611) -> (queue out=w623:refnum<queue>)  [unwired: 1 in, 2 out]
      }
      event "Start": Value Change {
        n259 = event-data() -> ()  [unwired: 1 in, 2 out]
        n260 = Enqueue Element At Opposite End(queue=w629, element=T12 {"State"=enum."Open", "Para."=variant}) -> (queue out=w628:refnum<queue>)  [unwired: 2 in, 2 out]
      }
      event "m/z (Da)", "Integration Width (±Da)": Value Change {
        n261 = event-data() -> ()  [unwired: 1 in, 2 out]
        n262 = Enqueue Element(queue=w631, element=T12 {"State"=enum."Refresh_Profile", "Para."=variant}) -> (queue out=w630:refnum<queue>)  [unwired: 2 in, 2 out]
      }
      event "SaveMiddleFile": Value Change {
        n263 = event-data() -> ()  [unwired: 1 in, 6 out]
        n264 = Enqueue Element(queue=w635, element=T12 {"State"=enum."SaveMiddleFile", "Para."=variant}) -> (queue out=w634:refnum<queue>)  [unwired: 2 in, 2 out]
      }
      event "BinWidth", "#Layers", "Shot#": Value Change; "Spectra": Scale Range Change {
        n265 = event-data() -> ()  [unwired: 1 in, 1 out]
        n266 = Enqueue Element(queue=w640, element=T12 {"State"=enum."Refresh_Spectra", "Para."=variant}) -> ()  [unwired: 2 in, 3 out]
      }
      event "Depth Profile": Mouse Down {
        n267 = event-data() -> ("Coords"=w660:T23, "Mods.Double Click"=w643:bool, "Button"=w653:u16, "Coords.Horizontal"=w646:i32, "Coords.Vertical"=w645:i32)  [unwired: 1 in]
        n268 = control-ref of="Depth Profile"() -> (w652:refnum<vi>)
        n269 = case shown="1" w653 {
          frame Default {
          }
          frame 3 {
            # "middle"
          }
          frame 1 {
            # "left"
          }
          frame 2 {
            # "right"
          }
        }
        n270 = property on="Property Node" class="WFGraph (strict)"(reference=w652) -> (error out=w658:errorcluster, "ActXScl"=w655:i32, "ActYScl"=w656:i32, "Plot Bounds"=w651:T24)  [unwired: 1 in, 1 out]
        n271 = Unbundle By Name(w651) -> ("Right"=w650:i16, "Left"=w649:i16, "Bottom"=w648:i16, "Top"=w647:i16)
        n272 = invoke on="Invoke Node" class="WFGraph (strict)" method="Map Coords To XY"(reference=w652, error in=w658, "Coords"=w660, "X Scale"=w655, "Y Scale"=w656) -> ("XY"=w657:cluster{"X":dbl, "Y":dbl})  [unwired: 2 in, 6 out]
        n273 = In Range and Coerce(upper limit=w650, x=w646, lower limit=w649) -> (In Range?=w642:bool)  [unwired: 1 out]
        n274 = In Range and Coerce(upper limit=w648, x=w645, lower limit=w647) -> (In Range?=w641:bool)  [unwired: 1 out]
        n275 = Unbundle By Name(w657) -> ("X"=w654:dbl)
        n276 = Compound Arithmetic op=AND(w643, w642, w641) -> (w644:bool)
        n277 = case shown="True" w644 {
          tunnel: w654 -> [_ w662]
          frame False {
          }
          frame True {
            n278 = property on="Shot#" class="DigNum (strict)"("Val(Sgnl)"=w662) -> ()  [unwired: 2 in, 2 out]
          }
        }
      }
      event "Spectra": Mouse Down {
        n279 = event-data() -> ("Coords"=w682:T23, "Mods.Double Click"=w664:bool, "Button"=w676:u16, "Coords.Horizontal"=w666:i32, "Coords.Vertical"=w665:i32)  [unwired: 1 in]
        n280 = case shown="Default" w676 {
          frame Default {
          }
          frame 3 {
            # "middle"
          }
          frame 1 {
            # "left"
          }
          frame 2 {
            # "right"
          }
        }
        n281 = property on="Property Node" class="XYGraph (strict)"(reference=w675) -> (error out=w680:errorcluster, "ActXScl"=w677:i32, "ActYScl"=w678:i32, "Plot Bounds"=w667:T24)  [unwired: 1 in, 1 out]
        n282 = Unbundle By Name(w667) -> ("Right"=w673:i16, "Left"=w672:i16, "Bottom"=w671:i16, "Top"=w670:i16)
        n283 = invoke on="Invoke Node" class="XYGraph (strict)" method="Map Coords To XY"(reference=w675, error in=w680, "Coords"=w682, "X Scale"=w677, "Y Scale"=w678) -> ("XY"=w679:cluster{"X":dbl, "Y":dbl})  [unwired: 2 in, 6 out]
        n284 = In Range and Coerce(upper limit=w673, x=w666, lower limit=w672) -> (In Range?=w669:bool)  [unwired: 1 out]
        n285 = In Range and Coerce(upper limit=w671, x=w665, lower limit=w670) -> (In Range?=w668:bool)  [unwired: 1 out]
        n286 = Compound Arithmetic op=AND(w664, w669, w668) -> (w663:bool)
        n287 = Unbundle By Name(w679) -> ("X"=w674:dbl)
        "m/z" <- w674
        n288 = case shown="True" w663 {
          tunnel: w674 -> [_ w684]
          frame False {
          }
          frame True {
            n289 = property on="m/z (Da)" class="DigNum (strict)"("Val(Sgnl)"=w684) -> ()  [unwired: 2 in, 2 out]
          }
        }
      }
      event "Fullscale X": Value Change {
        n290 = event-data() -> ()  [unwired: 1 in, 1 out]
        n291 = property class="XYGraph (strict)"(reference=w687) -> (reference out=w694:refnum<vi>, "Value"=w691:cluster{"Array":dbl[], dbl[]})  [unwired: 1 in, 1 out]
        n292 = Unbundle(w691) -> ("Array"=w692:dbl[])  [unwired: 1 out]
        n293 = control-ref of="BinWidth"() -> (w686:refnum<vi>)
        n294 = Array Max & Min(array=w692) -> (max value=w693:dbl, min value=w688:dbl)  [unwired: 2 out]
        n295 = property class="DigNum (strict)"(reference=w686) -> (reference out=w695:refnum<vi>, "Value"=w696:dbl)  [unwired: 1 in, 1 out]
        n296 = In Range and Coerce(upper limit=w693, x=0.0 ("X Scale.Range:Minimum"), lower limit=w688) -> (coerced(x)=w690:dbl)  [unwired: 1 out]
        n297 = property on="Property Node" class="XYGraph (strict)"(reference=w694, "XScale.Maximum"=w693, "XScale.Minimum"=w690) -> (error out=w697:errorcluster)  [unwired: 1 in, 1 out]
        n298 = property class="DigNum (strict)"(reference=w695, error in=w697, "Val(Sgnl)"=w696) -> ()  [unwired: 2 out]
      }
      event "Fullscale Y": Value Change {
        n299 = event-data() -> ()  [unwired: 1 in, 1 out]
        n300 = call-poly "Autoscale_Y.vi"("GraphRef"=w700) -> ()  [unwired: 11 in]
      }
      event "Linear/Log": Value Change {
        n301 = event-data() -> ()  [unwired: 1 in, 1 out]
        n302 = Select(t=u8 1 ("Y Scale.Mapping Mode"), s="Linear/Log", f=u8 0 ("Y Scale.Mapping Mode")) -> (s? t:f=w702:u8)
        n303 = property on="Spectra" class="XYGraph (strict)"("YScale.Mapping Mode"=w702) -> ()  [unwired: 2 in, 2 out]
      }
      event "X++": Value Change {
        n304 = event-data() -> ()  [unwired: 1 in, 1 out]
        n305 = property on="Property Node" class="XYGraph (strict)"(reference=w710) -> (reference out=w721:refnum<vi>, "XScale.Maximum"=w720:dbl, "XScale.Minimum"=w719:dbl)  [unwired: 1 in, 1 out]
        n306 = Add(x=w720, y=w719) -> (x+y=w718:dbl)
        n307 = Subtract(x=w720, y=w719) -> (x-y=w715:dbl)
        n308 = Multiply(x=0.5, y=w718) -> (x*y=w714:dbl)
        n309 = Multiply(x=0.25, y=w715) -> (x*y=w713:dbl)
        n310 = control-ref of="BinWidth"() -> (w709:refnum<vi>)
        n311 = Add(x=w714, y=w713) -> (x+y=w712:dbl)
        n312 = Subtract(x=w714, y=w713) -> (x-y=w711:dbl)
        n313 = property class="DigNum (strict)"(reference=w709) -> (reference out=w722:refnum<vi>, "Value"=w723:dbl)  [unwired: 1 in, 1 out]
        n314 = property on="Property Node" class="XYGraph (strict)"(reference=w721, "XScale.Maximum"=w712, "XScale.Minimum"=w711) -> (error out=w724:errorcluster)  [unwired: 1 in, 1 out]
        n315 = property class="DigNum (strict)"(reference=w722, error in=w724, "Val(Sgnl)"=w723) -> ()  [unwired: 2 out]
      }
      event "X--": Value Change {
        n316 = event-data() -> ()  [unwired: 1 in, 1 out]
        n317 = property on="Property Node" class="XYGraph (strict)"(reference=w728) -> (reference out=w739:refnum<vi>, "XScale.Maximum"=w738:dbl, "XScale.Minimum"=w737:dbl)  [unwired: 1 in, 1 out]
        n318 = control-ref of="BinWidth"() -> (w727:refnum<vi>)
        n319 = Add(x=w738, y=w737) -> (x+y=w736:dbl)
        n320 = Subtract(x=w738, y=w737) -> (x-y=w733:dbl)
        n321 = Multiply(x=0.5, y=w736) -> (x*y=w732:dbl)
        n322 = Multiply(x=1.0, y=w733) -> (x*y=w731:dbl)
        n323 = Add(x=w732, y=w731) -> (x+y=w730:dbl)
        n324 = Subtract(x=w732, y=w731) -> (x-y=w729:dbl)
        n325 = property class="DigNum (strict)"(reference=w727) -> (reference out=w740:refnum<vi>, "Value"=w742:dbl)  [unwired: 1 in, 1 out]
        n326 = property on="Property Node" class="XYGraph (strict)"(reference=w739, "XScale.Maximum"=w730, "XScale.Minimum"=w729) -> (error out=w741:errorcluster)  [unwired: 1 in, 1 out]
        n327 = property class="DigNum (strict)"(reference=w740, error in=w741, "Val(Sgnl)"=w742) -> ()  [unwired: 2 out]
      }
      event "Y--": Value Change {
        n328 = event-data() -> ()  [unwired: 1 in, 1 out]
        n329 = property on="Property Node" class="XYGraph (strict)"(reference=w745) -> (reference out=w764:refnum<vi>, "Value"=w763:cluster{"Array":dbl[], dbl[]}, "XScale.Maximum"=w751:dbl, "XScale.Minimum"=w752:dbl, "YScale.Maximum"=w760:dbl, "YScale.Minimum"=w761:dbl)  [unwired: 1 in, 1 out]
        n330 = Unbundle(w763) -> ("Array"=w749:dbl[], w750:dbl[])
        n331 = for {
          tunnel: w750 -> [w767] mode=indexing
          tunnel: w749 -> [w771] mode=indexing
          tunnel: w752 -> [w770]
          tunnel: w751 -> [w769]
          tunnel: [w766] -> w753 mode=indexing
          n332 = In Range and Coerce(upper limit=w769, x=w771, lower limit=w770) -> (In Range?=w768:bool)  [unwired: 1 out]
          n333 = case shown="True" w768 {
            tunnel: w767 -> [_ w772]
            tunnel: [_ w772] -> w766
            frame False {
              (unwired) nan
            }
            frame True {
            }
          }
        }
        n334 = Array Max & Min(array=w753) -> (min value=w759:dbl)  [unwired: 3 out]
        n335 = In Range and Coerce(upper limit=w760, x=w759, lower limit=w761) -> (coerced(x)=w762:dbl)  [unwired: 1 out]
        n336 = Subtract(x=w760, y=w762) -> (x-y=w754:dbl)
        n337 = Subtract(x=w762, y=w761) -> (x-y=w756:dbl)
        n338 = Multiply(x=2.0, y=w754) -> (x*y=w747:dbl)
        n339 = Multiply(x=2.0, y=w756) -> (x*y=w757:dbl)
        n340 = Add(x=w762, y=w747) -> (x+y=w748:dbl)
        n341 = Subtract(x=w762, y=w757) -> (x-y=w758:dbl)
        n342 = property on="Property Node" class="XYGraph (strict)"(reference=w764, "YScale.Maximum"=w748, "YScale.Minimum"=w758) -> ()  [unwired: 1 in, 2 out]
      }
      event "Y++": Value Change {
        n343 = event-data() -> ()  [unwired: 1 in, 1 out]
        n344 = property on="Property Node" class="XYGraph (strict)"(reference=w774) -> (reference out=w793:refnum<vi>, "Value"=w792:cluster{"Array":dbl[], dbl[]}, "XScale.Maximum"=w780:dbl, "XScale.Minimum"=w781:dbl, "YScale.Maximum"=w789:dbl, "YScale.Minimum"=w790:dbl)  [unwired: 1 in, 1 out]
        n345 = Unbundle(w792) -> ("Array"=w778:dbl[], w779:dbl[])
        n346 = for {
          tunnel: w779 -> [w796] mode=indexing
          tunnel: w778 -> [w800] mode=indexing
          tunnel: w781 -> [w799]
          tunnel: w780 -> [w798]
          tunnel: [w795] -> w782 mode=indexing
          n347 = In Range and Coerce(upper limit=w798, x=w800, lower limit=w799) -> (In Range?=w797:bool)  [unwired: 1 out]
          n348 = case shown="True" w797 {
            tunnel: w796 -> [_ w801]
            tunnel: [_ w801] -> w795
            frame False {
              (unwired) nan
            }
            frame True {
            }
          }
        }
        n349 = Array Max & Min(array=w782) -> (min value=w788:dbl)  [unwired: 3 out]
        n350 = In Range and Coerce(upper limit=w789, x=w788, lower limit=w790) -> (coerced(x)=w791:dbl)  [unwired: 1 out]
        n351 = Subtract(x=w789, y=w791) -> (x-y=w783:dbl)
        n352 = Subtract(x=w791, y=w790) -> (x-y=w785:dbl)
        n353 = Multiply(x=0.5, y=w783) -> (x*y=w776:dbl)
        n354 = Multiply(x=0.5, y=w785) -> (x*y=w786:dbl)
        n355 = Add(x=w791, y=w776) -> (x+y=w777:dbl)
        n356 = Subtract(x=w791, y=w786) -> (x-y=w787:dbl)
        n357 = property on="Property Node" class="XYGraph (strict)"(reference=w793, "YScale.Maximum"=w777, "YScale.Minimum"=w787) -> ()  [unwired: 1 in, 2 out]
      }
    }
    "UserEventIter." <- w556
  }
  n358 = Release Queue "Release Queue\nAfter all quit."(queue=w12, error in (no error)=w14) -> (error out=→"error out":errorcluster)  [unwired: 1 in, 2 out]
